vi "Set TDF File.vi"(8 "error in (no error)":errorcluster caption="에러 입력(에러 없음)", 10 "TDF File Name":string, 11 "Instrument Manager 입력":refnum<class "Instrument Manager.lvclass">) -> (0 "error out":errorcluster caption="에러 출력", 3 "Instrument Manager 출력":refnum<class "Instrument Manager.lvclass">)   [LabVIEW 2023, in "Instrument Manager.lvclass"]
uses:
  Instrument Manager.lvclass
  Instrument Manager.lvclass/Instrument Manager.ctl
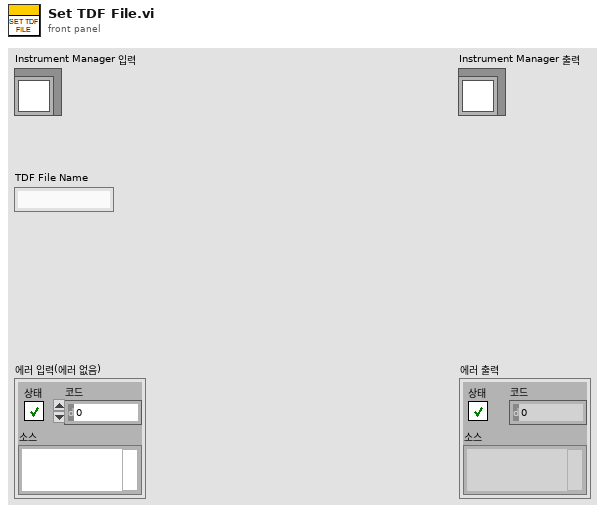
[diagram p1: front panel]
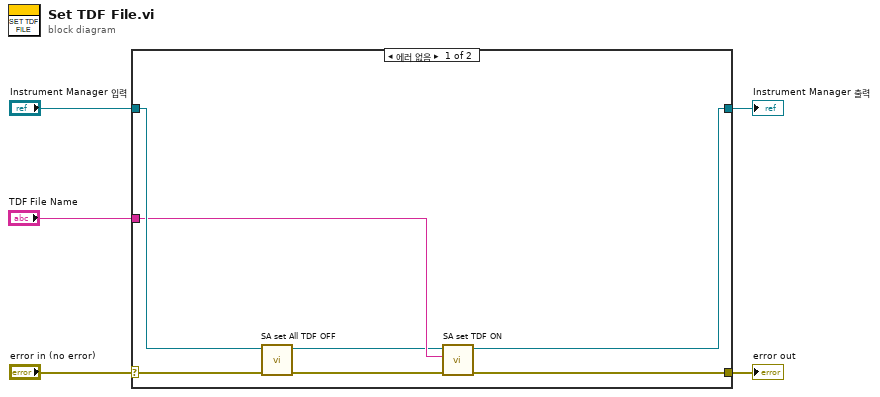
[diagram p0: block diagram]
diagram:
  n1 = case shown="에러 없음" "error in (no error)" {
    selector: "error in (no error)" -> [w11 w14]
    tunnel: [w8 w14] -> w4
    tunnel: [w6 w13] -> w2
    tunnel: "Instrument Manager 입력" -> [w12 w13]
    tunnel: "TDF File Name" -> [w10 _]
    frame No Error {
      n2 = call "SA set All TDF OFF.vi"("error in (no error)"=w11, "Instrument Manager 입력"=w12) -> ("error out"=w9:errorcluster, "Instrument Manager 출력"=w7:refnum<class "Instrument Manager.lvclass">)  [unwired: 8 in]
      n3 = call "SA set TDF ON.vi"("error in (no error)"=w9, "TDF File Name"=w10, "Instrument Manager 입력"=w7) -> ("error out"=w8:errorcluster, "Instrument Manager 출력"=w6:refnum<class "Instrument Manager.lvclass">)  [unwired: 7 in]
    }
    frame Error {
    }
  }
  "error out" <- w4
  "Instrument Manager 출력" <- w2
